vi "GDSLvIcon_CreateIconPicture.vi"(1 "FrameColor":u32(colorbox), 2 "FrameThickness(1)":u32=1, 3 "HeaderIconIn":u8[][](array[numeric]) format="%x", 4 "BodyIconIn":u8[][](array[numeric]) format="%x", 5 "error in (no error)":errorcluster, 6 "ImageRows(32)":i32=32, 7 "BigSizeIcon(x6)":i32=6, 8 "RowStart(0)":i32, 9 "BgIcon":T1 {"ColorsOkayforiconToBeOnTopOf" format="%x"}, 11 "0px Splitter(False)":bool) -> (13 "BodyIconOut":u8[][](array[numeric]) format="%x", 15 "WholeIconOut":u8[][](array[numeric]) format="%x", 16 "IconPictureOut":picture, 17 "LargeIconPictureOut(x6)":picture, 18 "BodyOffset":cluster{"X":i32, "Y":i32}, 19 "error out":errorcluster)   [LabVIEW 2020]
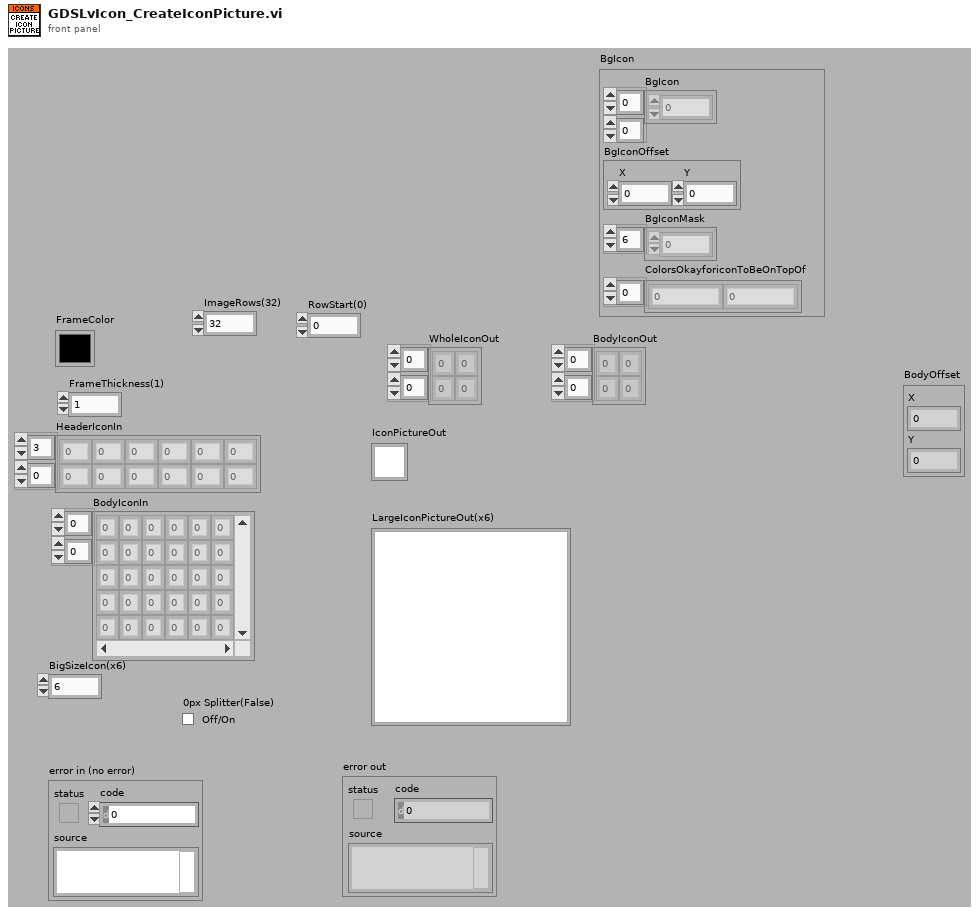
[diagram p1: front panel]
types:
  T1 = cluster{"BgIcon":u8[][], "BgIconOffset":cluster{"X":i32, "Y":i32}, "BgIconMask":u8[], "ColorsOkayforiconToBeOnTopOf":u8[]}
  T2 = cluster{"left":i16, "top":i16, "right":i16, "bottom":i16}
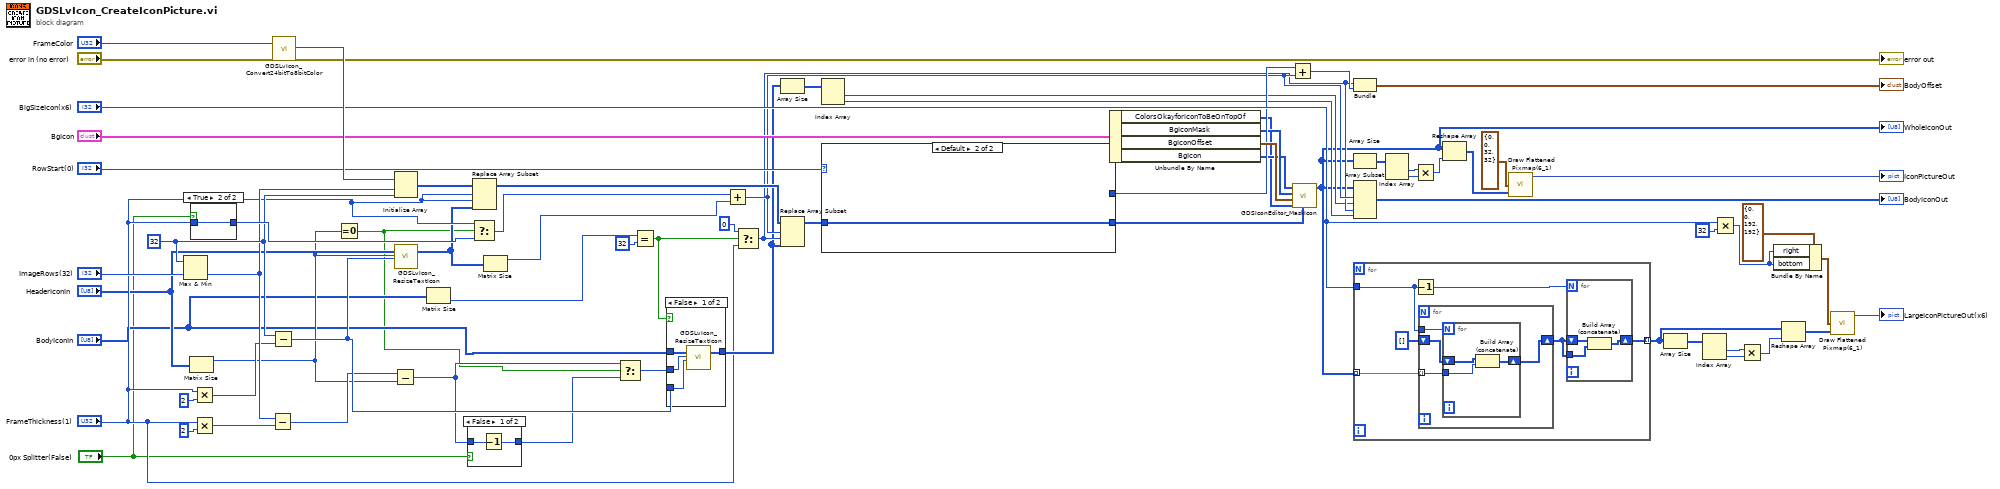
[diagram p0: block diagram]
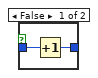
[diagram p3: hidden frame]
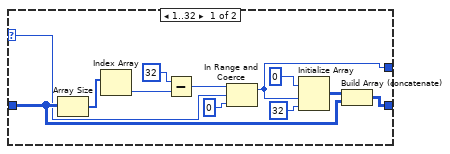
[diagram p4: hidden frame]
diagram:
  w26 = 32 ("dimension size")
  n1 = Max & Min(x=w26, y="ImageRows(32)") -> (min(x,y)=w25:i32)  [unwired: 1 out]
  n2 = Matrix Size(0:"HeaderIconIn") -> (1:w8:i32)  [unwired: 1 out]
  n3 = case shown="True" "0px Splitter(False)" {
    tunnel: [w72 w73] -> w42
    tunnel: "FrameThickness(1)" -> [w71 w73]
    frame False {
      n4 = Increment(x=w71) -> (x+1=w72:u32)
    }
    frame True {
    }
  }
  n5 = Multiply(x="FrameThickness(1)", y=u32 2) -> (x*y=w11:u32)
  n6 = Multiply(x="FrameThickness(1)", y=u32 2) -> (x*y=w10:u32)
  n7 = Subtract(x=w25, y=w10) -> (x-y=w36:u32)
  n8 = Subtract(x=w26, y=w11) -> (x-y=w50:u32)
  n9 = call <resource>:"GDSLvIcon_Convert24bitTo8bitColor.vi"("Color 24bit In"="FrameColor", "error in (no error)"="error in (no error)") -> ("Color out(256)"=w68:u8, "error out"=→"error out":errorcluster)  [unwired: 14 in, 2 out]
  n10 = Equal To 0?(x=w8) -> (x = 0?=w3:bool)
  n11 = Subtract(x=w36, y=w8) -> (x-y=w44:u32)
  n12 = Initialize Array(w68, w25, w26) -> (w67:u8[][])
  n13 = call <resource>:"GDSLvIcon_ResizeTextIcon.vi"("IconIn"="HeaderIconIn", "Rows/Height"=w8, "Columns/Width"=w50) -> ("IconOut"=w5:u8[][])  [unwired: 15 in, 1 out]
  n14 = Matrix Size(0:"BodyIconIn") -> (2:w6:i32)  [unwired: 1 out]
  n15 = case shown="False" "0px Splitter(False)" {
    tunnel: [w75 w76] -> w45
    tunnel: w44 -> [w74 w76]
    frame False {
      n16 = Decrement(x=w74) -> (x-1=w75:u32)
    }
    frame True {
    }
  }
  n17 = Select(t="FrameThickness(1)", s=w3, f=w42) -> (s? t:f=w41:u32)
  n18 = Replace Array Subset(array=w67, new element=w5, index (row)="FrameThickness(1)", index (col)="FrameThickness(1)") -> (w66:u8[][])
  n19 = Matrix Size(0:w5) -> (1:w4:i32)  [unwired: 1 out]
  n20 = Select(t=w44, s=w3, f=w45) -> (s? t:f=w43:u32)
  n21 = Equal?(x=w6, y=32) -> (x = y?=w38:bool)
  n22 = case shown="False" w38 {
    tunnel: [w80 w81] -> w22
    tunnel: w50 -> [w79 _]
    tunnel: w43 -> [w78 _]
    tunnel: "BodyIconIn" -> [w77 w81]
    frame False {
      n23 = call <resource>:"GDSLvIcon_ResizeTextIcon.vi"("IconIn"=w77, "Rows/Height"=w78, "Columns/Width"=w79) -> ("IconOut"=w80:u8[][])  [unwired: 15 in, 1 out]
    }
    frame True {
    }
  }
  n24 = Add(x=w41, y=w4) -> (x+y=w24:u32)
  n25 = Select(t=u32 0, s=w38, f="FrameThickness(1)") -> (s? t:f=w23:u32)
  n26 = Array Size(array=w22) -> (size(s)=w21:i32[])
  n27 = Replace Array Subset(array=w66, new element=w22, index (row)=w24, index (col)=w23) -> (w34:u8[][])
  n28 = Index Array(array=w21) -> (element #1=w20:i32, element #2=w19:i32)  [unwired: 2 in]
  n29 = case shown="Default" "RowStart(0)" {
    selector: "RowStart(0)" -> [w83 _]
    tunnel: [w90 w94] -> w33
    tunnel: w34 -> [w89 w94]
    tunnel: [w82 _] -> w30
    frame 1..32 {
      n30 = Array Size(array=w89) -> (size(s)=w88:i32[])
      n31 = Index Array(array=w88) -> (element=w86:i32)  [unwired: 1 in]
      n32 = Subtract(x=32 ("dimension size"), y=w86) -> (x-y=w84:i32)
      n33 = In Range and Coerce(upper limit=w84, x=w83, lower limit=0) -> (coerced(x)=w82:i32)  [unwired: 1 out]
      n34 = Initialize Array(u8 0 ("element"), w82, 32 ("dimension size")) -> (w91:u8[][])
      n35 = Build Array (concatenate)(w91, w89) -> (w90:u8[][])
    }
    frame Default {
    }
  }
  n36 = Unbundle By Name("BgIcon") -> ("ColorsOkayforiconToBeOnTopOf"=w14:u8[], "BgIconMask"=w17:u8[], "BgIconOffset"=w31:cluster{"X":i32, "Y":i32}, "BgIcon"=w15:u8[][])
  n37 = Add(x=w30, y=w24) -> (x+y=w28:u32)
  n38 = call <resource>:"GDSIconEditor_MaskIcon.vi"("BgIcon"=w33, "ColorsOkayforiconToBeOnTopOf"=w14, "BgIconOffset"=w31, "BgIconMask"=w17, "IconIn"=w15) -> ("IconOut"=w16:u8[][])  [unwired: 6 in]
  "WholeIconOut" <- w16
  n39 = Bundle("FrameThickness(1)"=w23, w28) -> (→"BodyOffset":cluster{"FrameThickness(1)":u32, u32})  [unwired: 1 in]
  n40 = Array Size(array=w16) -> (size(s)=w53:i32[])
  n41 = Array Subset(array=w16, index (row)=w24, length (row)=w20, index (col)=w23, length (col)=w19) -> (→"BodyIconOut":u8[][])
  n42 = for {
    tunnel: w16 -> [w100] mode=indexing
    tunnel: [w98] -> w60 mode=indexing
    tunnel: "BigSizeIcon(x6)" -> [w95]
    n43 = Decrement(x=w95) -> (x-1=w96:i32)
    n44 = for {
      tunnel: w100 -> [w107] mode=indexing
      shift-right: [w105] -> w97
      shift-left: u8[] [] -> [w106]
      tunnel: w95 -> [w104]
      n45 = for {
        N: w104 -> [_]
        tunnel: w107 -> [w110]
        shift-right: [w108] -> w105
        shift-left: w106 -> [w109]
        n46 = Build Array (concatenate)(w109, w110) -> (w108:u8[])
      }
    }
    n47 = for {
      N: w96 -> [_]
      tunnel: w97 -> [w103]
      shift-right: [w101] -> w98
      shift-left: w97 -> [w102]
      n48 = Build Array (concatenate)(w102, w103) -> (w101:u8[])
    }
  }
  n49 = Index Array(array=w53) -> (element #1=w55:i32, element #2=w54:i32)  [unwired: 2 in]
  n50 = Multiply(x=w55, y=w54) -> (x*y=w56:i32)
  n51 = Reshape Array(w16, w56) -> (w57:u8[])
  n52 = call <vilib>:"Draw Flattened Pixmap(6_1).vi"("rect"=T2 {"left"=0, "top"=0, "right"=32, "bottom"=32}, "flattened pixmap data"=w57) -> ("new picture"=→"IconPictureOut":picture)  [unwired: 7 in]
  n53 = Array Size(array=w60) -> (size(s)=w64:i32[])
  n54 = Index Array(array=w64) -> (element #1=w62:i32, element #2=w63:i32)  [unwired: 2 in]
  n55 = Multiply(x="BigSizeIcon(x6)", y=32) -> (x*y=w46:i32)
  n56 = Multiply(x=w62, y=w63) -> (x*y=w61:i32)
  n57 = Bundle By Name(cluster=T2 {"left"=0, "top"=0, "right"=192, "bottom"=192} ("rect"), "right"=w46, "bottom"=w46) -> (w48:T2)
  n58 = Reshape Array(w60, w61) -> (w59:u8[])
  n59 = call <vilib>:"Draw Flattened Pixmap(6_1).vi"("rect"=w48, "flattened pixmap data"=w59) -> ("new picture"=→"LargeIconPictureOut(x6)":picture)  [unwired: 7 in]
